vi "shear_and_recovery_points_calculation__3e535a12e3.vi"(6 "stop steps":i32, 8 "loop period (ms)":dbl, 9 "# periods":dbl, 10 "recovery phase":dbl, 11 "frequency":dbl) -> (1 "Time needed":dbl, 2 "shear+stop points":dbl, 3 "shear points":dbl)   [LabVIEW 2023]
panel:
  out "recovery phase points":dbl
  out "x+y":dbl
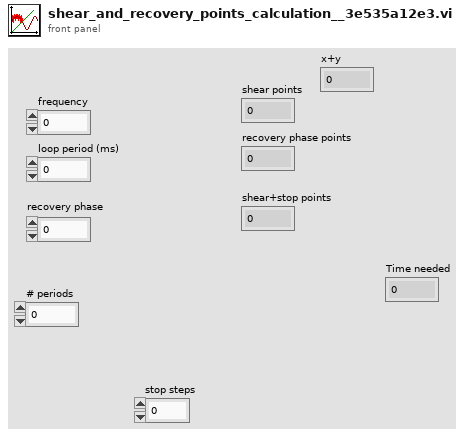
[diagram p1: front panel]
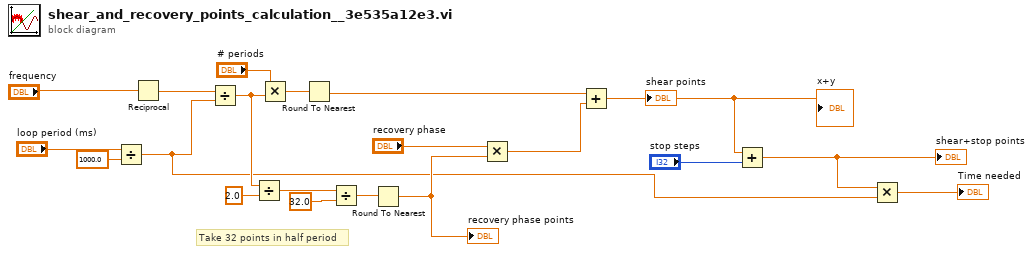
[diagram p0: block diagram]
diagram:
  # "Take 32 points in half period"
  n1 = Divide(x="loop period (ms)", y=1000.0) -> (x/y=w2:dbl)
  n2 = Reciprocal(x="frequency") -> (1/x=w16:dbl)
  n3 = Divide(x=w16, y=w2) -> (x/y=w12:dbl)
  n4 = Divide(x=w12, y=2.0) -> (x/y=w10:dbl)
  n5 = Multiply(x="# periods", y=w12) -> (x*y=w20:dbl)
  n6 = Round To Nearest(number=w20) -> (nearest integer value=w4:dbl)
  n7 = Divide(x=w10, y=32.0) -> (x/y=w8:dbl)
  n8 = Round To Nearest(number=w8) -> (nearest integer value=w6:dbl)
  "recovery phase points" <- w6
  n9 = Multiply(x="recovery phase", y=w6) -> (x*y=w5:dbl)
  n10 = Add(x=w4, y=w5) -> (x+y=w18:dbl)
  "shear points" <- w18
  "x+y" <- w18
  n11 = Add(x=w18, y="stop steps") -> (x+y=w3:dbl)
  "shear+stop points" <- w3
  n12 = Multiply(x=w3, y=w2) -> (x*y=→"Time needed":dbl)
